vi "Set Logger Enqueuer.vi"(8 "error in":errorcluster, 10 "Logger":refnum<class "Message Enqueuer.lvclass">, 11 "File Manager in":refnum<class "File Manager.lvclass">) -> (0 "error out":errorcluster, 3 "File Manager out":refnum<class "File Manager.lvclass">)   [LabVIEW 2026, in "File Manager.lvclass"]
doc: "Set the logger enqueuer for a Logger Client."
uses:
  File Manager.lvclass
  <vilib>/ActorFramework/Message Enqueuer/Message Enqueuer.lvclass
  File Manager.lvclass/File Manager.ctl
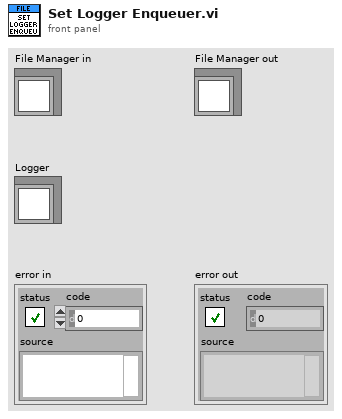
[diagram p1: front panel]
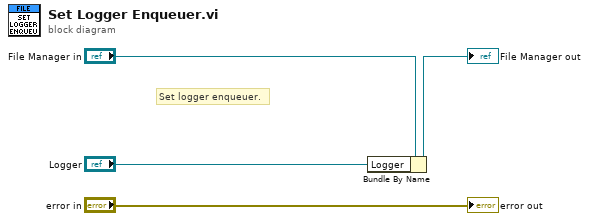
[diagram p0: block diagram]
diagram:
  # "Set logger enqueuer."
  n1 = Bundle By Name(cluster="File Manager in", "Logger"="Logger") -> (→"File Manager out":refnum<class "File Manager.lvclass">)
  "error out" <- "error in"
